vi "Lint VIs.vi"(8 "error in":errorcluster, 11 "Runner in":refnum<class "Runner.lvclass">) -> (0 "error out":errorcluster, 3 "Runner out":refnum<class "Runner.lvclass">)   [LabVIEW 2026, in "Runner.lvlib" / "Runner.lvclass"]
doc: "Lint all created VIs."
uses:
  Runner.lvclass
  Runner.lvclass/Runner.ctl
  Interfaces/ILogger/ILogger Messages/Log Msg/Log Msg.lvclass/Log Msg.ctl
  <vilib>/ActorFramework/Message Enqueuer/Message Enqueuer.lvclass/Message Enqueuer.ctl
  <vilib>/ActorFramework/Message Enqueuer/Enqueue.vi
  Interfaces/ILogger/ILogger Messages/Log Msg/Log Msg.lvclass
  <vilib>/ActorFramework/Message Priority Queue/Priority Enqueue.vi
  Interfaces/IProject Manager/IProject Manager.lvclass
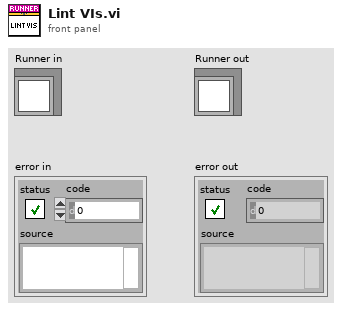
[diagram p1: front panel]
types:
  T1 = typedef "Log Entry--cluster.ctl" = cluster{"Time":timestamp, "Message":string}
  T2 = typedef "lib_blue_core.lvlib/API.lvclass/Options--cluster.ctl" = cluster{"Force?":bool, "Ignore List":string[], "Only List":string[], "Save(T)?":bool}
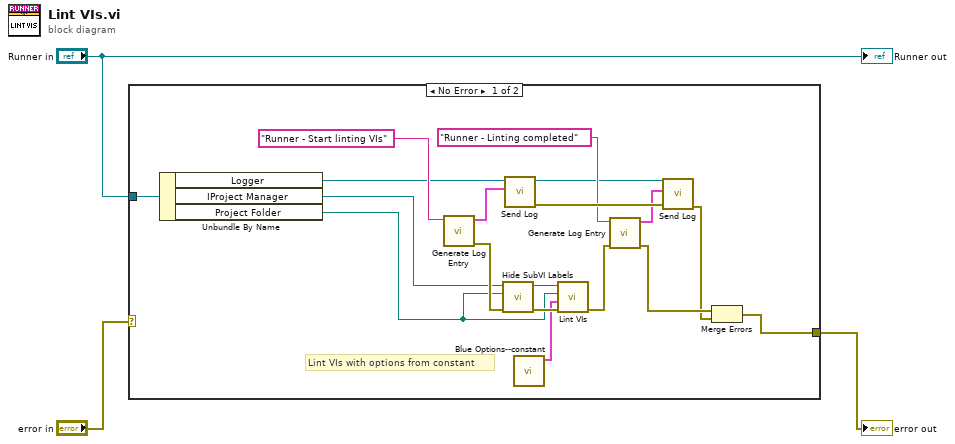
[diagram p0: block diagram]
diagram:
  n1 = case shown="No Error" "error in" {
    selector: "error in" -> [_ w22]
    tunnel: "Runner in" -> [w9 _]
    tunnel: [w17 w22] -> w2
    frame No Error {
      # "Lint VIs with options from constant"
      n2 = Unbundle By Name(w9) -> ("Logger"=w8:refnum<class "Message Enqueuer.lvclass">, "IProject Manager"=w7:refnum<class "IProject Manager.lvclass">, "Project Folder"=w5:path)
      n3 = call "Generate Log Entry.vi"("Message"="Runner - Start linting VIs") -> ("error out"=w16:errorcluster, "Log Entry"=w13:T1)  [unwired: 9 in]
      n4 = call-dynamic "Hide SubVI Labels.vi"("error in"=w16, "Project Root Folder"=w5, "IProject Manager in"=w7) -> ("error out"=w15:errorcluster, "IProject Manager out"=w6:refnum<class "IProject Manager.lvclass">)  [unwired: 7 in]
      n5 = call "Send Log.vi"("Log Entry"=w13, "Message Enqueuer"=w8) -> ("error out"=w21:errorcluster, "Message Enqueuer out"=w10:refnum<class "Message Enqueuer.lvclass">)  [unwired: 8 in]
      n6 = call "Blue Options--constant.vi"() -> ("Options"=w4:T2)  [unwired: 11 in]
      n7 = call-dynamic "Lint VIs.vi"("error in"=w15, "Options"=w4, "Project Root Folder"=w5, "IProject Manager in"=w6) -> ("error out"=w20:errorcluster)  [unwired: 6 in, 1 out]
      n8 = call "Generate Log Entry.vi"("error in"=w20, "Message"="Runner - Linting completed") -> ("error out"=w19:errorcluster, "Log Entry"=w11:T1)  [unwired: 8 in]
      n9 = call "Send Log.vi"("error in (no error)"=w21, "Log Entry"=w11, "Message Enqueuer"=w10) -> ("error out"=w18:errorcluster)  [unwired: 7 in, 1 out]
      n10 = Merge Errors(w19, w18) -> (w17:errorcluster)
    }
    frame Error {
      # "Pass error without further action."
    }
  }
  "error out" <- w2
  "Runner out" <- "Runner in"
